vi "Host_Exit.vi"(8 "error in":errorcluster, 9 "Camera":refnum<k5>, 10 "Motion":refnum<visa-resource-name>, 11 "Lot No":string) -> (3 "error out":errorcluster)   [LabVIEW 2018]
doc: "Use this template to build a VI to use as a subVI."
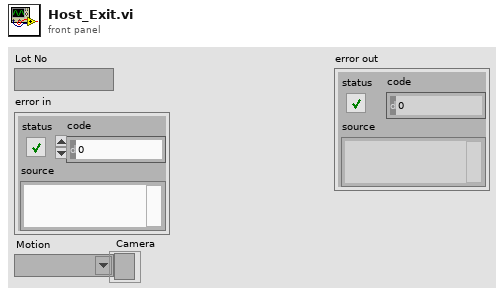
[diagram p1: front panel]
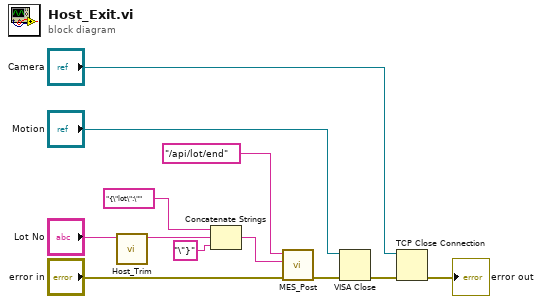
[diagram p0: block diagram]
diagram:
  n1 = call "Host_Trim.vi"("string"="Lot No") -> ("trimmed string"=w10:string)  [unwired: 10 in]
  n2 = Concatenate Strings("{\"lot\":\"", w10, "\"}") -> (w8:string)
  n3 = call "MES_Post.vi"("error in (no error)"="error in", "Body"=w8, "Path"="/api/lot/end") -> ("error out"=w4:errorcluster)  [unwired: 5 in, 3 out]
  n4 = VISA Close(VISA resource name="Motion", error in (no error)=w4) -> (error out=w2:errorcluster)
  n5 = TCP Close Connection(connection ID="Camera", error in (no error)=w2) -> (error out=→"error out":errorcluster)  [unwired: 1 in, 1 out]
